vi "Remove Item From Group.vi"(8 "error in (no error)":errorcluster, 11 "Selector in":refnum<class "Selector.lvclass">) -> (0 "error out":errorcluster, 2 "Name":string, 3 "Selector out":refnum<class "Selector.lvclass">)   [LabVIEW 2019, in "Selector.lvclass"]
uses:
  Selector.lvclass
  Selector.lvclass/Selector.ctl
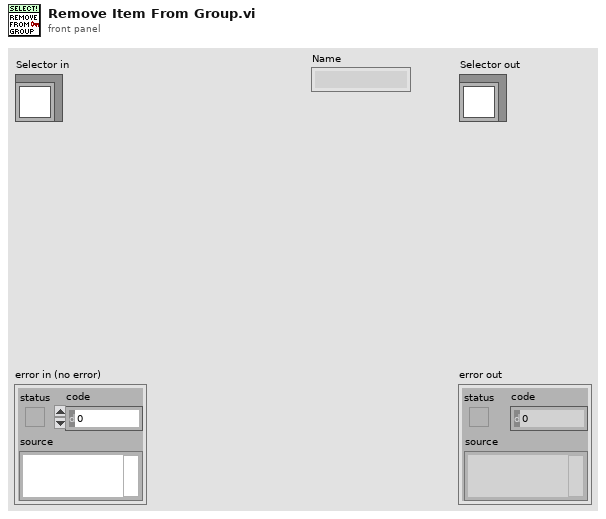
[diagram p1: front panel]
types:
  T1 = typedef "Selector.lvclass/Item.ctl" = cluster{"Name":string, "Group":string, "Enabled":bool}
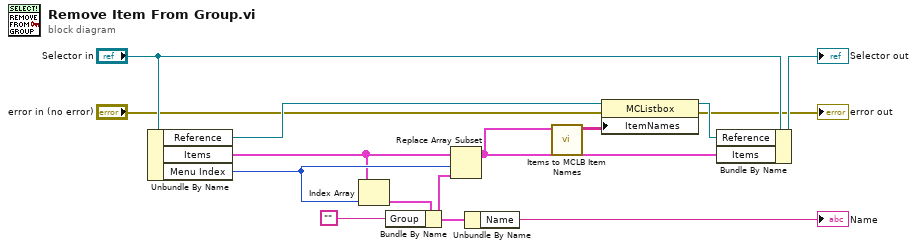
[diagram p0: block diagram]
diagram:
  n1 = Unbundle By Name("Selector in") -> ("Reference"=w12:refnum<vi>, "Items"=w3:T1[], "Menu Index"=w6:i32)
  n2 = Index Array(array=w3, index=w6) -> (element=w8:T1)
  n3 = Bundle By Name(cluster=w8, "Group"="") -> (w2:T1)
  n4 = Replace Array Subset(array=w3, new element=w2, index=w6) -> (w4:T1[])
  n5 = Unbundle By Name(w2) -> ("Name"=→"Name":string)
  n6 = call "Items to MCLB Item Names.vi"("Items"=w4) -> ("Item Names"=w5:string[][])  [unwired: 6 in]
  n7 = property class="MCListbox"(reference=w12, error in="error in (no error)", "ItemNames"=w5) -> (reference out=w11:refnum<vi>, error out=→"error out":errorcluster)
  n8 = Bundle By Name(cluster="Selector in", "Reference"=w11, "Items"=w4) -> (→"Selector out":refnum<class "Selector.lvclass">)
